vi "test Digital Pattern Output.vi"(8 "error in (no error)":errorcluster, 11 "TestCase in":refnum<class "Engine Simulation IO System Tests.lvclass">) -> (0 "error out":errorcluster, 3 "TestCase out":refnum<class "Engine Simulation IO System Tests.lvclass">)   [LabVIEW 2020, in "Engine Simulation IO System Tests.lvclass"]
uses:
  Engine Simulation IO System Tests.lvclass
  C:/Program Files (x86)/National Instruments/LabVIEW 2020/vi.lib/NI/VeriStand Custom Device Testing Tools/VeriStandTestCase/VeriStandTestCase.lvclass
  Engine Simulation IO System Tests.lvclass/Engine Simulation IO System Tests.ctl
  <vilib>/NI/LVFPGA Adv Session Resources/OpenByNameSubVI.vi
  <vilib>/NI VeriStand/Execution/Workspace/NI VeriStand - Set Single Channel Value.vi
  <vilib>/rvi/interface/common/dynamic/niFpgaEscapeDelimiterAndNull.vi
  <vilib>/Utility/error.llb/Error Cluster From Error Code.vi
  <vilib>/rvi/errors/niLvFpgaAdjustHostInterfaceError.vi
  <vilib>/FPGAPlugInAG/Dynamic/niLvFpga_Close_Dynamic.vi
  <vilib>/NI/LVFPGA Adv Session Resources/OpenByName.xnode
  <vilib>/rvi/interface/nirviReadWriteControl/nirviReadWriteControl.xnode
  <vilib>/rvi/interface/nirviCloseFPGA/nirviCloseFPGA.xnode
  <vilib>/addons/_JKI Toolkits/VI Tester/TestCase.llb/TestCase.lvclass
  <vilib>/NI VeriStand/Execution/Workspace/NI_VS Workspace ExecutionAPI.lvlib
  System Explorer/Digital Pattern Find Events Enum.ctl
  System Explorer/Engine Simulation Toolkit System Explorer.lvlib
  NiFpgaLv.dll
  <vilib>/rvi/interface/Simulation/niFpgaSimulationCallBeginRW.vi
  System Explorer/Digital Pattern Add Pulse.ctl
  System Explorer/Digital Pattern Remove Edge.ctl
  System Explorer/Digital Pattern Base.ctl
  System Explorer/Digital Pattern.ctl
  <vilib>/NI/LVFPGA Adv Session Resources/LVFPGAAdvSessionResources.lvlib
  C:/Program Files (x86)/National Instruments/LabVIEW 2020/vi.lib/addons/_JKI Toolkits/VI Tester/TestCase.llb/TestCase.lvclass
panel:
  out "Values":T1(array[cluster])
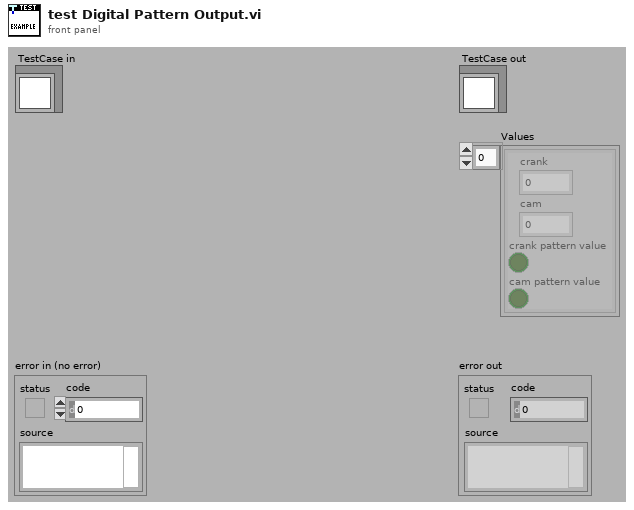
[diagram p1: front panel]
types:
  T1 = cluster{"crank":u16, "cam":u16, "crank pattern value":bool, "cam pattern value":bool}[]
  T2 = typedef "Engine Simulation Toolkit System Explorer.lvlib/Digital Pattern.ctl" = cluster{"Name":string, "Base":T3, "Remove":T4[], "Add":T5[], "FPGA Resource":string}
  T3 = typedef "Engine Simulation Toolkit System Explorer.lvlib/Digital Pattern Base.ctl" = cluster{"Length":dbl, "Teeth":u16, "Width":dbl, "Offset":dbl}
  T4 = typedef "Engine Simulation Toolkit System Explorer.lvlib/Digital Pattern Remove Edge.ctl" = cluster{"Tooth":u16, "Edge":bool}
  T5 = typedef "Engine Simulation Toolkit System Explorer.lvlib/Digital Pattern Add Pulse.ctl" = cluster{"Tooth":u16, "Offset":dbl, "Width":dbl}
  T6 = typedef "Engine Simulation Toolkit System Explorer.lvlib/Digital Pattern Find Events Enum.ctl" = enum16{"Rising Edge", "Falling Edge", "Any Edge", "Center Tooth", "Center Gap"}
  T7 = cluster{"Name":string, "Depth":u32, "Write? (Deprecated:Use Implementation)":bool, "Physical Channel":u32, "Base Address":u32, "Data Width":u32, "Data Type":enum32{"Boolean", "I8", "I16", "I32", "I64", "U8", "U16", "U32", "U64", "FXP", "CustomControl", "SGL"}, "FXP Properties":variant, "Write Window Address":u32, "Implementation":enum16{"niFpgaTargetToHost", "niFpgaHostToTarget", "niFpgaPeerToPeerWriter", "niFpgaPeerToPeerReader", "niCoreTargetToHost", "niCoreHostToTarget"}, "Control Set":u32}[]
  T8 = cluster{"Name":string, "type":variant, "indicator?":bool}[]
  T9 = typedef "NI_VS Workspace ExecutionAPI.lvlib/WorkspaceAPI.ctl" = refnum<k24>
  T10 = typedef "Engine Simulation Toolkit System Explorer.lvlib/Digital Pattern Expanded.ctl" = cluster{"X":dbl[], "Y":dbl[]}
  T11 = cluster{"crank":u16, "cam":u16, "crank pattern value":bool, "cam pattern value":bool}
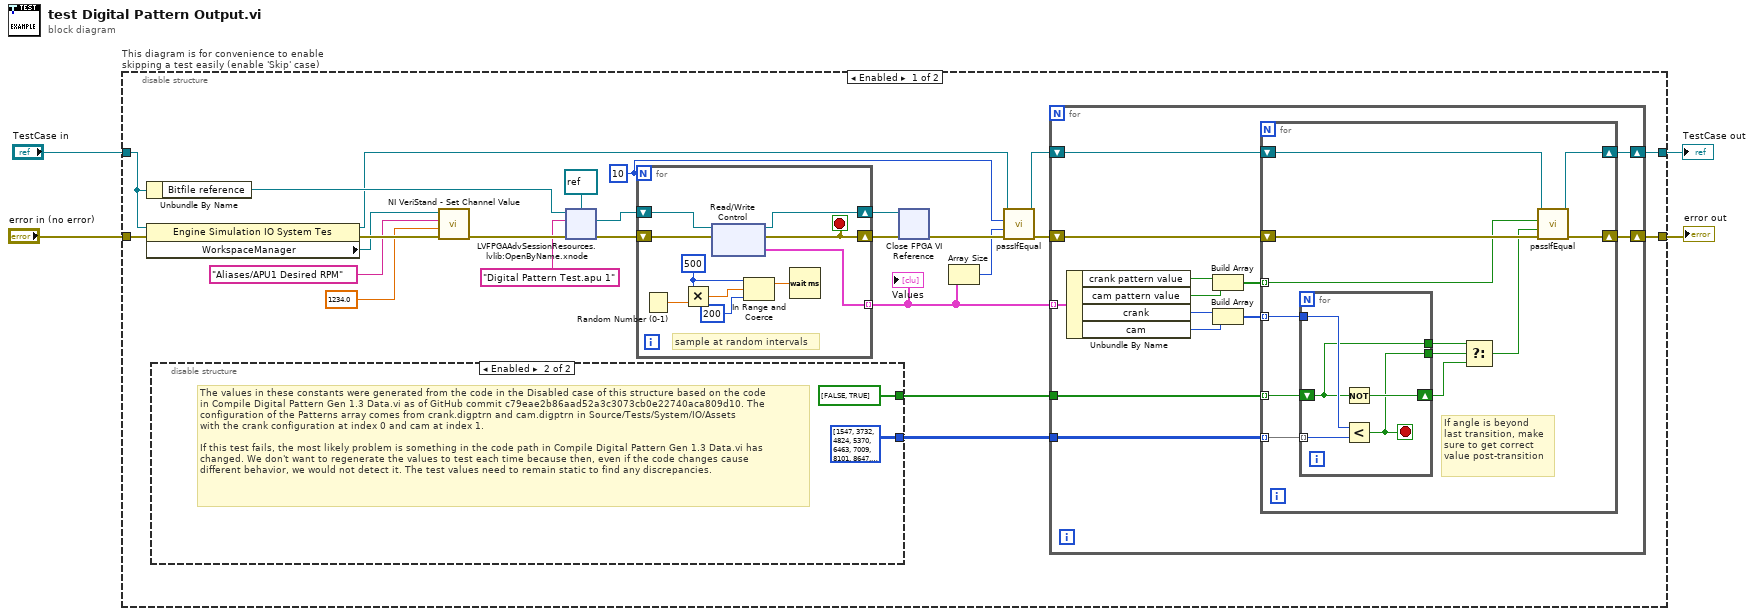
[diagram p0: block diagram]
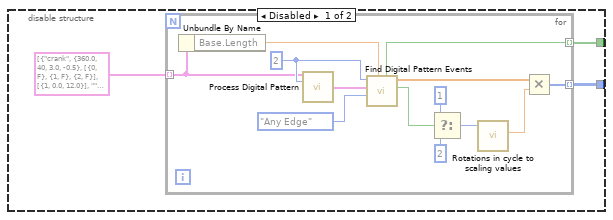
[diagram p2: hidden frame]
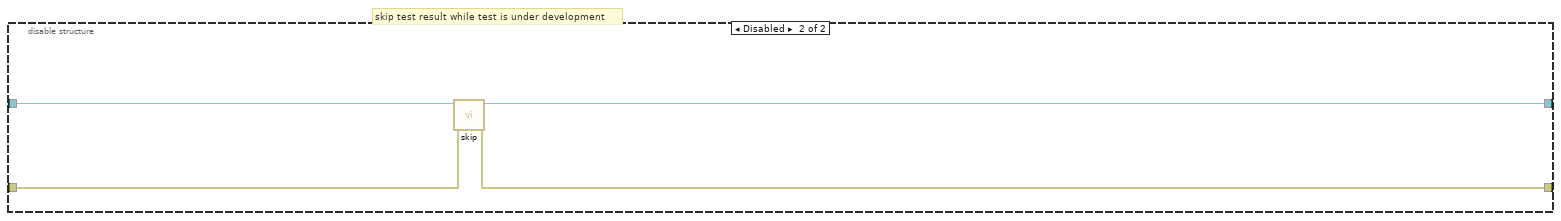
[diagram p3: hidden frame]
diagram:
  n1 = disable-structure "This diagram is for convenience to enable skipping a test easily (enable 'Skip' case)" shown="Enabled" {
    disable-tunnel: "TestCase in" -> [w14 w104]
    disable-tunnel: [w13 w102] -> w1
    disable-tunnel: [w12 w103] -> w3
    disable-tunnel: "error in (no error)" -> [w29 w101]
    frame Enabled {
      w7 = 10
      n2 = Unbundle By Name(w14) -> ("Bitfile reference"=w23:refnum<k20>)
      n3 = property class="Engine Simulation IO System Tes"(reference=w14, error in=w29) -> (reference out=w6:refnum<class "Engine Simulation IO System Tests.lvclass">, error out=w28:errorcluster, "WorkspaceManager"=w27:T9)
      n4 = disable-structure shown="Enabled" {
        disable-tunnel: [w32 bool[] [FALSE, TRUE] ("First Falling")] -> w16
        disable-tunnel: [w31 u16[][] [[1547, 3732, 4824, 5370, 6463, 7009, 8101, 8647, 9739, 10286, 11378, 11924, 13016, 13562, 14655, 15201, 16293, 16839, 17931, 18478, 19570, 20116, 21208, 21754, 22847, 23393, 24485, 25031, 26123, 26670, 27762, 28308, 29400, 29946, 31039, 31585, 32677, 33223, 34315, 34862, 35954, 36500, 37592, 38138, 39231, 39777, 40869, 41415, 42507, 43054, 44146, 44692, 45784, 46330, 47423, 47969, 49061, 49607, 50699, 51246, 52338, 52884, 53976, 54522, 55615, 56161, 57253, 57799, 58891, 59438, 60530, 61076, 62168, 62714, 63807, 64353], [4506, 13062, 17613, 26169, 30720, 39276, 43827, 52383, 56934, 65490, 0, 0, 0, 0, 0, 0, 0, 0, 0, 0, 0, 0, 0, 0, 0, 0, 0, 0, 0, 0, 0, 0, 0, 0, 0, 0, 0, 0, 0, 0, 0, 0, 0, 0, 0, 0, 0, 0, 0, 0, 0, 0, 0, 0, 0, 0, 0, 0, 0, 0, 0, 0, 0, 0, 0, 0, 0, 0, 0, 0, 0, 0, 0, 0, 0, 0]] ("Position LUT")] -> w15
        frame Disabled {
          n5 = for {
            tunnel: T2[] [{"Name"="crank", "Base"={"Length"=360.0, "Teeth"=40, "Width"=3.0, "Offset"=-0.5}, "Remove"=[{"Tooth"=0, "Edge"=FALSE}, {"Tooth"=1, "Edge"=FALSE}, {"Tooth"=2, "Edge"=FALSE}], "Add"=[{"Tooth"=1, "Offset"=0.0, "Width"=12.0}], "FPGA Resource"=""}, {"Name"="cam", "Base"={"Length"=720.0, "Teeth"=5, "Width"=50.0, "Offset"=-0.5}, "Remove"=[], "Add"=[], "FPGA Resource"=""}] ("Patterns") -> [w42] mode=indexing
            tunnel: [w39] -> w31 mode=indexing
            tunnel: [w33] -> w32 mode=indexing
            w44 = u16 2 ("Rotations")
            n6 = Unbundle By Name(w42) -> ("Base.Length"=w34:dbl)
            n7 = call "Process Digital Pattern.vi"("EPT Pattern"=w42, "Rotations"=w44) -> ("Final"=w45:T10)  [unwired: 7 in, 6 out]
            n8 = call "Find Digital Pattern Events.vi"("Base.length"=w34, "Event"=Digital_Pattern_Find_Events_Enum."Any Edge", "Pattern"=w45, "Rotations"=w44) -> ("crank angle"=w36:bool, "Locations"=w41:dbl[], "first falling"=w33:bool)  [unwired: 5 in]
            n9 = Select(t=u16 1 ("Rotations"), s=w36, f=u16 2 ("Rotations")) -> (s? t:f=w35:u16)
            n10 = call "Rotations in cycle to scaling values.vi"("rotations in a cycle"=w35) -> ("angle to u16 scale factor"=w40:dbl)  [unwired: 8 in, 2 out]
            n11 = Multiply(x=w41, y=w40) -> (x*y=w39:u16[])
          }
        }
        frame Enabled {
          # "The values in these constants were generated from the code in the Disabled case of this structure based on the code\nin Compile Digital Pattern Gen 1.3 Data.vi as of GitHub commit c79eae2b86aad52a3c3073cb0e22740aca809d10. The\nconfiguration of the Patterns array comes from crank.digptrn and cam.digptrn in Source/Tests/System/IO/Assets\nwith the crank configuration at index 0 and cam at index 1.\n\nIf this test fails, the most likely problem is something in the code path in Compile Digital Pattern Gen 1.3 Data.vi has\nchanged. We don't want to regenerate the values to test each time because then, even if the code changes cause\ndifferent behavior, we would not detect it. The test values need to remain static to find any discrepancies."
        }
      }
      n12 = call-poly <vilib>:"NI VeriStand - Set Channel Value.vi"("error in (no error)"=w28, "Value"=1234.0, "Channel"="Aliases/APU1 Desired RPM", "WorkspaceManager in"=w27) -> ("error out"=w24:errorcluster)  [unwired: 6 in, 1 out]
      n13 = xnode "LVFPGAAdvSessionResources.lvlib:OpenByName.xnode"("FPGA VI Reference in"=w23, "Resource name in"="Digital Pattern Test.apu 1", "Single resource reference type in"=refnum<k20> refnum, "Error in"=w24) -> ("Single resource reference out"=w19:refnum<k20>, "Error out"=w20:errorcluster)  [unwired: 1 out]
      n14 = for {
        N: w7 -> [_]
        shift-right: [w78] -> w18
        shift-left: w20 -> [w87]
        shift-right: [w85] -> w17
        shift-left: w19 -> [w86]
        tunnel: [w84] -> w9 mode=indexing
        stop <- w78 stop-if-true
        w82 = u32 500 ("milliseconds to wait")
        # "sample at random intervals"
        n15 = Random Number (0-1)() -> (number: 0 to 1=w83:dbl)
        n16 = Multiply(x=w82, y=w83) -> (x*y=w81:dbl)
        n17 = xnode "Read/Write Control"("FPGA VI Reference In"=w86, "error in"=w87) -> ("FPGA VI Reference Out"=w85:refnum<k20>, "error out"=w78:errorcluster, "Value"=w84:T11)
        n18 = In Range and Coerce(upper limit=w82, x=w81, lower limit=u32 200 ("milliseconds to wait")) -> (coerced(x)=w79:dbl)  [unwired: 1 out]
        n19 = Wait (ms)(milliseconds to wait=w79) -> ()  [unwired: 1 out]
      }
      "Values" <- w9
      n20 = xnode "Close FPGA VI Reference"("FPGA VI Reference In"=w17, "error in"=w18) -> ("error out"=w11:errorcluster)
      n21 = Array Size(array=w9) -> (size(s)=w8:i32)
      n22 = call-dynamic "passIfEqual.vi"("error in (no error)"=w11, "y"=w8, "x"=w7, "TestCase in"=w6) -> ("error out"=w10:errorcluster, "TestCase out"=w5:refnum<class "Engine Simulation IO System Tests.lvclass">)  [unwired: 6 in]
      n23 = for {
        tunnel: w9 -> [w60] mode=indexing
        tunnel: w16 -> [w59]
        tunnel: w15 -> [w58]
        shift-right: [w53] -> w13
        shift-left: w5 -> [w54]
        shift-right: [w51] -> w12
        shift-left: w10 -> [w52]
        n24 = Unbundle By Name(w60) -> ("crank pattern value"=w50:bool, "cam pattern value"=w49:bool, "crank"=w57:u16, "cam"=w56:u16)
        n25 = Build Array(w50, w49) -> (w48:bool[])
        n26 = Build Array(w57, w56) -> (w55:u16[])
        n27 = for {
          tunnel: w59 -> [w71] mode=indexing
          tunnel: w58 -> [w72] mode=indexing
          tunnel: w55 -> [w66] mode=indexing
          shift-right: [w68] -> w53
          shift-left: w54 -> [w67]
          shift-right: [w69] -> w51
          shift-left: w52 -> [w70]
          tunnel: w48 -> [w62] mode=indexing
          # "If angle is beyond\nlast transition, make\nsure to get correct\nvalue post-transition"
          n28 = for {
            tunnel: w72 -> [w76] mode=indexing
            tunnel: w66 -> [w77]
            shift-right: [w75] -> w63
            shift-left: w71 -> [w74]
            tunnel: [w74] -> w64
            tunnel: [w73] -> w65
            stop <- w73 stop-if-true
            n29 = Not(x=w74) -> (.not. x?=w75:bool)
            n30 = Less?(x=w77, y=w76) -> (x < y?=w73:bool)
          }
          n31 = Select(t=w64, s=w65, f=w63) -> (s? t:f=w61:bool)
          n32 = call-dynamic "passIfEqual.vi"("error in (no error)"=w70, "y"=w61, "x"=w62, "TestCase in"=w67) -> ("error out"=w69:errorcluster, "TestCase out"=w68:refnum<class "Engine Simulation IO System Tests.lvclass">)  [unwired: 6 in]
        }
      }
    }
    frame Disabled {
      # "skip test result while test is under development"
      n33 = call <vilib>:"skip.vi"("error in (no error)"=w101, "TestCase in"=w104) -> ("error out"=w103:errorcluster, "TestCase out"=w102:refnum<class "Engine Simulation IO System Tests.lvclass">)  [unwired: 8 in]
    }
  }
  "error out" <- w3
  "TestCase out" <- w1
